vi "Get Service Class Instances.vi"() -> (3 "service instances":refnum<class "ServiceBase.lvclass">[](array[class]))   [LabVIEW 2020, in "thermal-chamber-controller_server.lvlib"]
uses:
  thermal-chamber-controller_server.lvlib
  <vilib>/gRPC/LabVIEW gRPC Servicer/ServiceBase/ServiceBase.lvclass
  RPC Service/ThermalChamberController/ThermalChamberController.lvclass
  C:/Program Files (x86)/National Instruments/LabVIEW 2020/vi.lib/gRPC/LabVIEW gRPC Servicer/ServiceBase/ServiceBase.lvclass
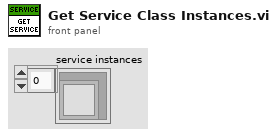
[diagram p1: front panel]
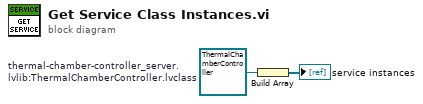
[diagram p0: block diagram]
diagram:
  w1 = refnum<class "ThermalChamberController.lvclass"> refnum  # thermal-chamber-controller_server.lvlib:ThermalChamberController.lvclass
  n1 = Build Array(w1) -> (→"service instances":refnum<class "ThermalChamberController.lvclass">[])
